vi "Write Device - Protocol.vi"(8 "error in (no error)":errorcluster, 10 "Device - Protocol":T1, 11 "LTE in":refnum<class "LTE.lvclass">) -> (0 "error out":errorcluster, 3 "LTE out":refnum<class "LTE.lvclass">)   [LabVIEW 2023, in "ANRITSU Call Box.lvlib" / "LTE.lvclass"]
uses:
  LTE.lvclass
  Type Definition/Call Device - Protocol Type Selector.ctl
  LTE.lvclass/LTE.ctl
  ANRITSU Call Box.lvlib
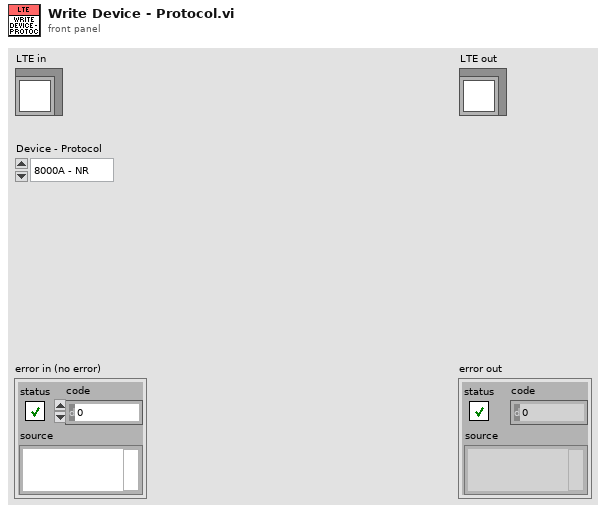
[diagram p1: front panel]
types:
  T1 = typedef "ANRITSU Call Box.lvlib/Call Device - Protocol Type Selector.ctl" = enum16{"8000A - NR", "8000A - LTE", "882xC - LTE"}
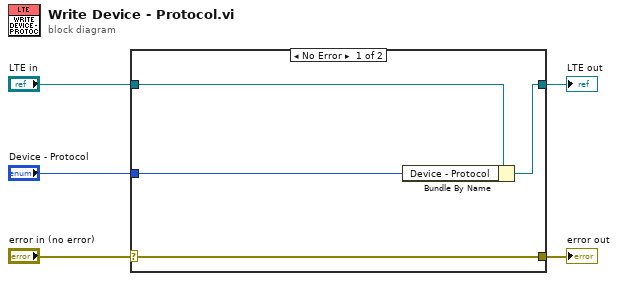
[diagram p0: block diagram]
diagram:
  n1 = case shown="No Error" "error in (no error)" {
    selector: "error in (no error)" -> [w9 w10]
    tunnel: [w9 w10] -> w4
    tunnel: [w7 w11] -> w2
    tunnel: "LTE in" -> [w8 w11]
    tunnel: "Device - Protocol" -> [w6 _]
    frame No Error {
      n2 = Bundle By Name(cluster=w8, "Device - Protocol"=w6) -> (w7:refnum<class "LTE.lvclass">)
    }
    frame Error {
    }
  }
  "error out" <- w4
  "LTE out" <- w2
